vi "SubSystems.vi"(8 "error in (no error)":errorcluster) -> ()   [LabVIEW 2027]
doc: "Start the robot subSystems that will run in parallel responding to commands sent by Auto and Tele OpModes.\nNewly scripted subSystems will be added automatically.\nIf subSystems aren't used, this is simply a home for a Periodic Task loop(s)."
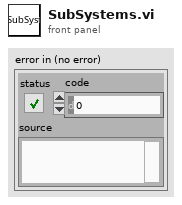
[diagram p1: front panel]
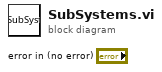
[diagram p0: block diagram]
diagram:
